vi "Send Request.vi"(6 "Reply?":bool, 8 "error in (no error)":errorcluster caption="错误输入（无错误）", 9 "Data输入":variant, 10 "命令":string, 11 "Queues":T1) -> (0 "error out":errorcluster caption="错误输出", 1 "有效?":bool, 2 "Data输出":variant)   [LabVIEW 2020, in "TCP Communication.lvlib"]
uses:
  TCP Communication.lvlib
  Reply.ctl
  Data Type.ctl
  Requset.ctl
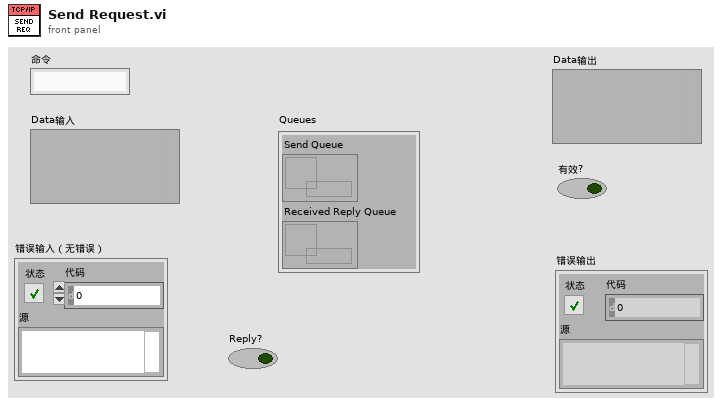
[diagram p1: front panel]
types:
  T1 = cluster{"Send Queue":refnum<queue>, "Received Reply Queue":refnum<queue>}
  T2 = typedef "TCP Communication.lvlib/Requset.ctl" = cluster{"ID":i32, "Reply?":bool, "CMD":string, "Data":variant}
  T3 = typedef "TCP Communication.lvlib/Data Type.ctl" = enum16{"Data Stream", "Status", "Request", "Reply"}
  T4 = typedef "TCP Communication.lvlib/Reply.ctl" = cluster{"ID":i32, "CMD":string, "Data":variant}
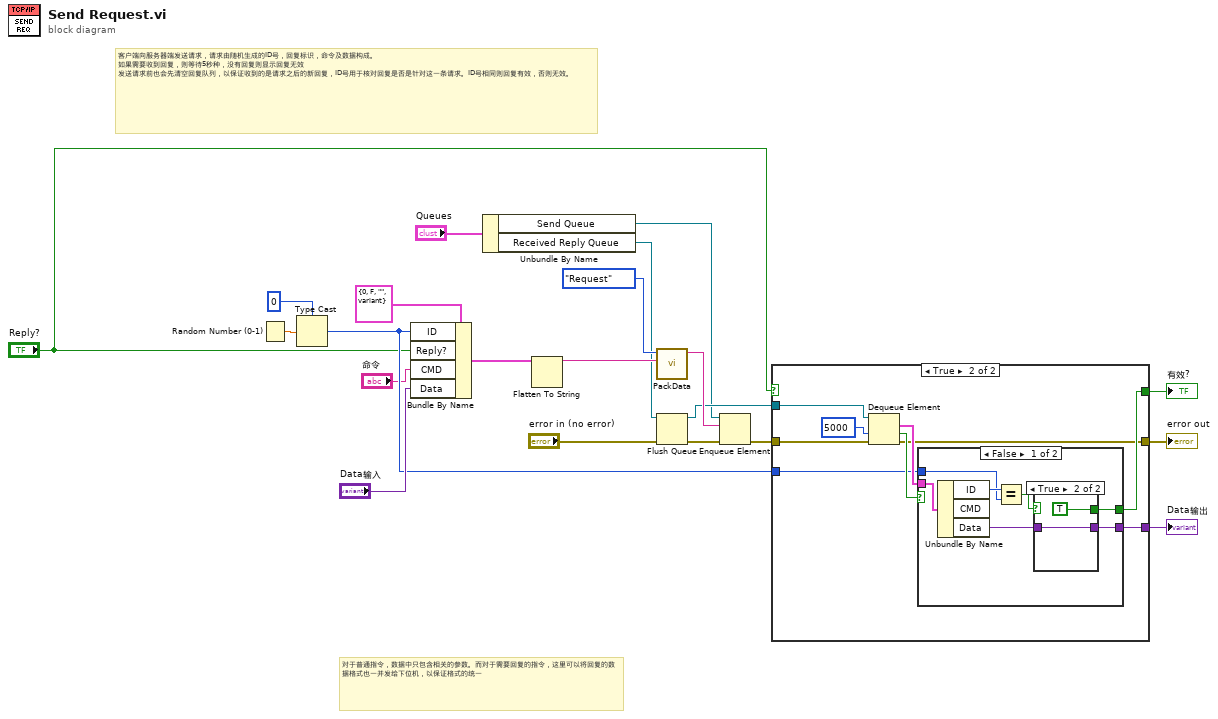
[diagram p0: block diagram]
diagram:
  # "对于普通指令，数据中只包含相关的参数。而对于需要回复的指令，这里可以将回复的数据格式也一并发给下位机，以保证格式的统一"
  # "客户端向服务器端发送请求，请求由随机生成的ID号，回复标识，命令及数据构成。\n如果需要收到回复，则等待5秒种，没有回复则显示回复无效\n发送请求前也会先清空回复队列，以保证收到的是请求之后的新回复，ID号用于核对回复是否是针对这一条请求。ID号相同则回复有效，否则无效。"
  n1 = Random Number (0-1)() -> (number: 0 to 1=w9:dbl)
  n2 = Type Cast(type=0, x=w9) -> (*(type *) &x=w18:i32)
  n3 = Bundle By Name(cluster=T2 {"ID"=0, "Reply?"=FALSE, "CMD"="", "Data"=variant} ("请求"), "ID"=w18, "Reply?"="Reply?", "CMD"="命令", "Data"="Data输入") -> (w13:T2)
  n4 = Unbundle By Name("Queues") -> ("Send Queue"=w2:refnum<queue>, "Received Reply Queue"=w1:refnum<queue>)
  n5 = Flatten To String(anything=w13) -> (data string=w15:string)  [unwired: 3 in, 2 out]
  n6 = call "PackData.vi"("字符串输入"=w15, "Data Type"=Data_Type."Request") -> ("字符串输出"=w16:string)  [unwired: 9 in]
  n7 = Flush Queue(queue=w1, error in (no error)="error in (no error)") -> (queue out=w4:refnum<queue>, error out=w5:errorcluster)  [unwired: 1 out]
  n8 = Enqueue Element(queue=w2, element=w16, error in (no error)=w5) -> (error out=w8:errorcluster)  [unwired: 1 in, 2 out]
  n9 = case shown="True" "Reply?" {
    tunnel: w4 -> [_ w31]
    tunnel: w18 -> [_ w27]
    tunnel: [_ w26] -> w19
    tunnel: [_ w25] -> w21
    tunnel: w8 -> [w22 w24]
    tunnel: [w22 w23] -> w7
    frame False {
    }
    frame True {
      n10 = Dequeue Element(queue=w31, timeout in ms (-1)=5000 ("超时毫秒(-1)"), error in (no error)=w24) -> (element=w28:T4, timed out?=w29:bool, error out=w23:errorcluster)  [unwired: 1 out]
      n11 = case shown="False" w29 {
        tunnel: w28 -> [w38 _]
        tunnel: w27 -> [w36 _]
        tunnel: [w33 _] -> w26
        tunnel: [w32 _] -> w25
        frame False {
          n12 = Unbundle By Name(w38) -> ("ID"=w37:i32, "Data"=w34:variant)  [unwired: 1 out]
          n13 = Equal?(x=w37, y=w36) -> (x = y?=w35:bool)
          n14 = case shown="True" w35 {
            tunnel: w34 -> [_ w40]
            tunnel: [_ w40] -> w33
            tunnel: [_ TRUE] -> w32
            frame False {
            }
            frame True {
            }
          }
        }
        frame True {
        }
      }
    }
  }
  "有效?" <- w21
  "Data输出" <- w19
  "error out" <- w7
